vi "SEPARAPALABRASPowerMeter.VI"(3 "error in":errorcluster, 4 "Comando":string, 5 "Tiempo de espera":u32=100, 6 "VISA resource name in":refnum<visa-resource-name>) -> (0 "error out":errorcluster, 1 "Salida":string, 2 "VISA resource name out":refnum<visa-resource-name>)   [LabVIEW 2020]
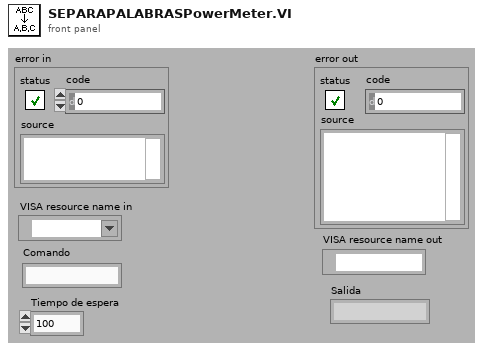
[diagram p1: front panel]
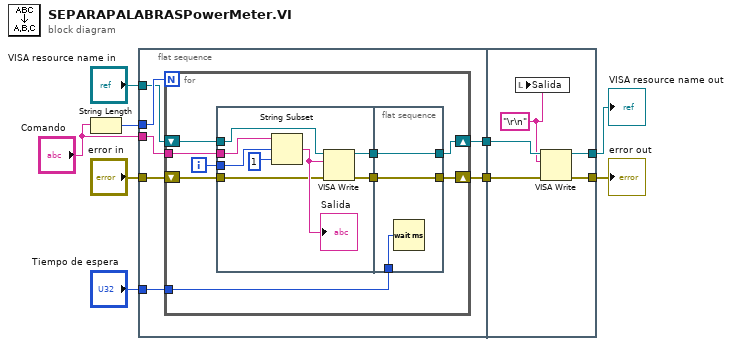
[diagram p0: block diagram]
diagram:
  n1 = String Length(string="Comando") -> (length=w9:i32)
  n2 = flat-sequence {
    tunnel: w9 -> [w16]
    tunnel: "VISA resource name in" -> [w15]
    tunnel: "Comando" -> [w14]
    tunnel: "Tiempo de espera" -> [w13]
    tunnel: "error in" -> [w12]
    tunnel: [w11] -> w3
    tunnel: [w10] -> w2
    tunnel: [w41] -> w5
    tunnel: w3 -> [w40]
    tunnel: w2 -> [w39]
    tunnel: [w38] -> w1
    frame #0 {
      n3 = for {
        N: w16 -> [_]
        tunnel: w14 -> [w23]
        tunnel: w13 -> [w22]
        shift-right: [w20] -> w11
        shift-left: w12 -> [w19]
        shift-right: [w17] -> w10
        shift-left: w15 -> [w25]
        i -> [w24]
        n4 = flat-sequence {
          tunnel: w25 -> [w33]
          tunnel: w24 -> [w32]
          tunnel: w23 -> [w30]
          tunnel: [w28] -> w21
          tunnel: w19 -> [w27]
          tunnel: [w26] -> w18
          tunnel: w22 -> [w36]
          tunnel: w21 -> [w35]
          tunnel: [w35] -> w20
          tunnel: [w34] -> w17
          tunnel: w18 -> [w34]
          frame #0 {
            n5 = String Subset(string=w30, offset (0)=w32, length (rest)=1 ("length (rest)")) -> (substring=w29:string)
            "Salida" <- w29
            n6 = VISA Write(VISA resource name=w33, write buffer=w29, error in (no error)=w27) -> (VISA resource name out=w26:refnum<visa-resource-name>, error out=w28:errorcluster)  [unwired: 1 out]
          }
          frame #1 {
            n7 = Wait (ms)(milliseconds to wait=w36) -> ()  [unwired: 1 out]
          }
        }
      }
    }
    frame #1 {
      w37 = "\r\n"
      n8 = local write "Salida"(w37) -> ()
      n9 = VISA Write(VISA resource name=w39, write buffer=w37, error in (no error)=w40) -> (VISA resource name out=w38:refnum<visa-resource-name>, error out=w41:errorcluster)  [unwired: 1 out]
    }
  }
  "error out" <- w5
  "VISA resource name out" <- w1
